vi "RemoteVI Send Windows.vi"(0 "clients":T1(array[cluster]), 5 "windows":T2(array[cluster]), 7 "message":string, 9 "capture?":bool) -> (4 "clients out":T1(array[cluster]))   [LabVIEW 2020, in "RemoteVI.lvlib"]
doc: "Sends the application's other windows to every client (docs\\protocol.md section 7): message (windows [...]) is encoded once as a WebSocket text frame, and when capture? is TRUE (a frame was made in this iteration, so windows follow the frame rate) every listed window is captured once (RemoteVI Capture Windows.vi). Then each client gets the list when it changed and each window's changes as a WINDOW FRAME (RemoteVI Send Client Windows.vi). No VI Server call."
uses:
  RemoteVI.lvlib
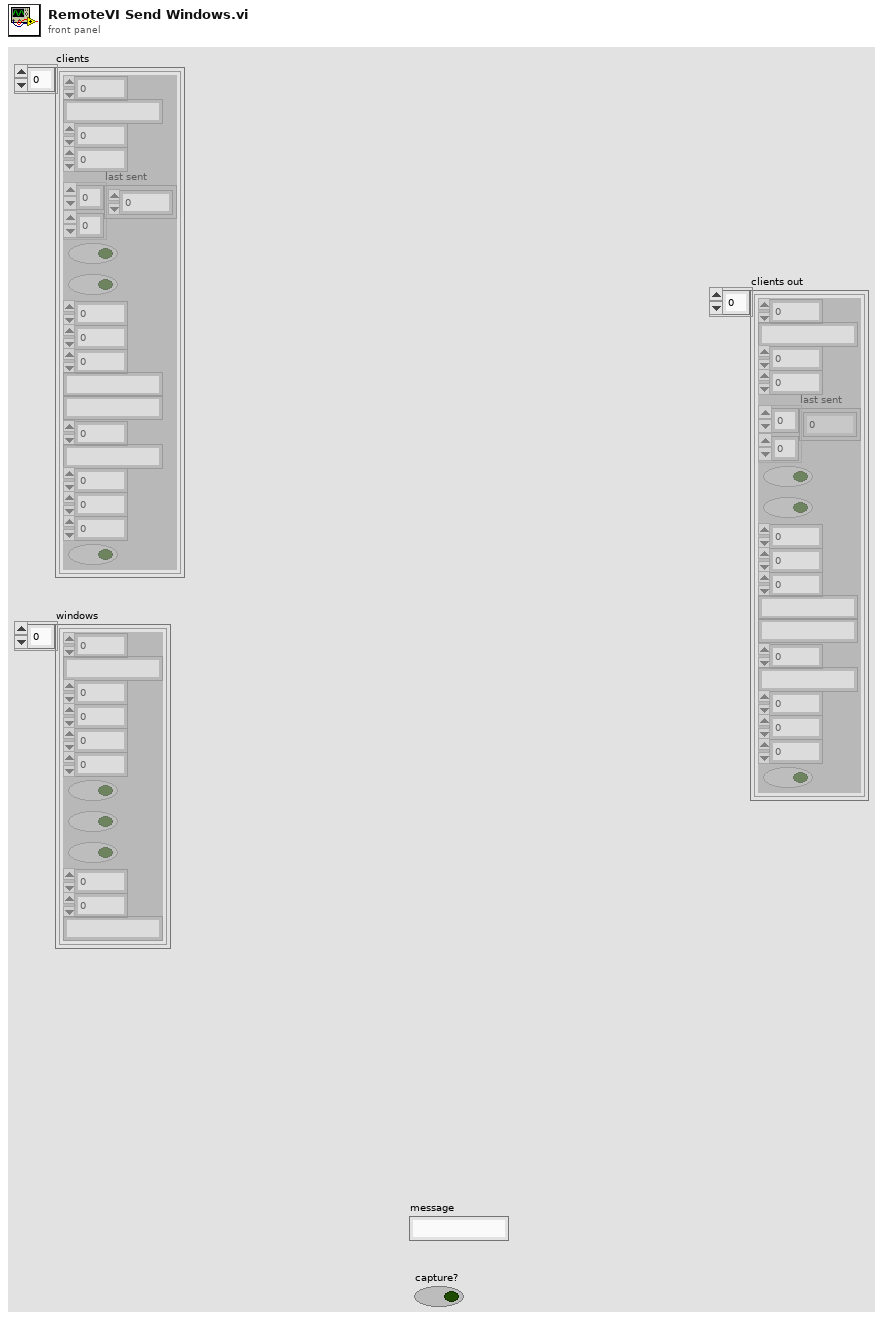
[diagram p1: front panel]
types:
  T1 = cluster{"connection":u32, "rx buffer":string, "seq":u32, "acked":u32, "last sent":u32[][], "tracking":bool, "closed":bool, "mods":u8, "mods set":u8, "popup since":u32, "windows sent":string, "window frames":cluster{"id":u64, "pixels":u32[][]}[], "key window":u64, "address":string, "since":dbl, "last input":dbl, "bytes":dbl, "view only":bool}[]
  T2 = cluster{"id":u64, "title":string, "x":i32, "y":i32, "w":i32, "h":i32, "modal":bool, "active":bool, "closable":bool, "sx":i32, "sy":i32, "class":string}[]
  T3 = cluster{"id":u64, "pixels":u32[][], "width":i32, "height":i32}[]
  T4 = cluster{"connection":u32, "rx buffer":string, "seq":u32, "acked":u32, "last sent":u32[][], "tracking":bool, "closed":bool, "mods":u8, "mods set":u8, "popup since":u32, "windows sent":string, "window frames":cluster{"id":u64, "pixels":u32[][]}[], "key window":u64, "address":string, "since":dbl, "last input":dbl, "bytes":dbl, "view only":bool}
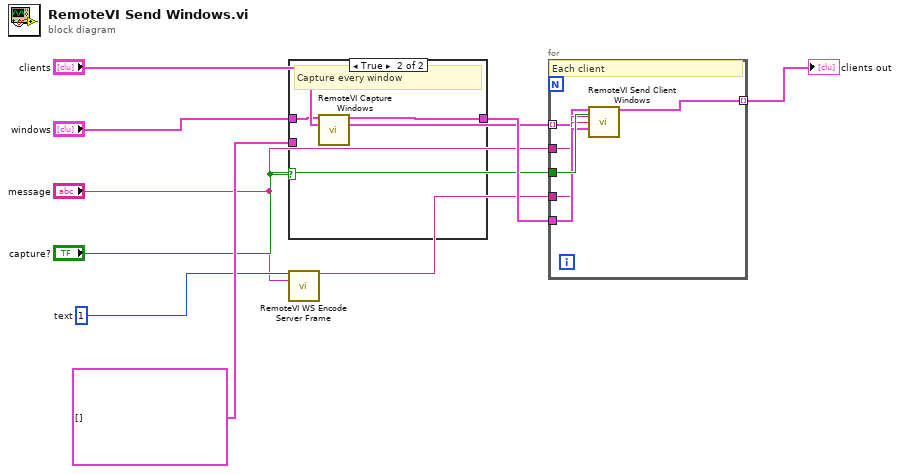
[diagram p0: block diagram]
diagram:
  w5 = u8 1  # text
  n1 = case shown="True" "capture?" {
    tunnel: "windows" -> [_ w11]
    tunnel: T3 [] -> [w10 _]
    tunnel: [w10 w12] -> w8
    frame False {
    }
    frame True {
      # "Capture every window"
      n2 = call "RemoteVI Capture Windows.vi"("windows"=w11) -> ("captures"=w12:T3)  [unwired: 14 in]
    }
  }
  n3 = call "RemoteVI WS Encode Server Frame.vi"("opcode"=w5, "payload"="message") -> ("frame"=w6:string)  [unwired: 13 in]
  n4 = for {
    tunnel: "clients" -> [w13] mode=indexing
    tunnel: "message" -> [w14]
    tunnel: "capture?" -> [w17]
    tunnel: w6 -> [w15]
    tunnel: w8 -> [w16]
    tunnel: [w18] -> w9 mode=indexing
    # "Each client"
    n5 = call "RemoteVI Send Client Windows.vi"("Client"=w13, "capture?"=w17, "message"=w14, "frame"=w15, "captures"=w16) -> ("Client out"=w18:T4)  [unwired: 10 in]
  }
  "clients out" <- w9
